vi "Test_C_RT_Path.vi"() -> ()   [LabVIEW 2021]
uses:
  CANsub_C.lvlib
  common/Typedefs/Bytes.ctl
  common/CANsub_Common.lvlib
  common/Typedefs/CAN_Frame.ctl
panel:
  out "ping length":i32
  out "encode mismatches":u32
  out "echo mismatches":u32
  out "error out":errorcluster
  out "peer close":bool
  out "decode errors":i32
  out "crc errors":u32
  out "frame mismatches":u32
  out "frames":i32
  # "Expected result when run"
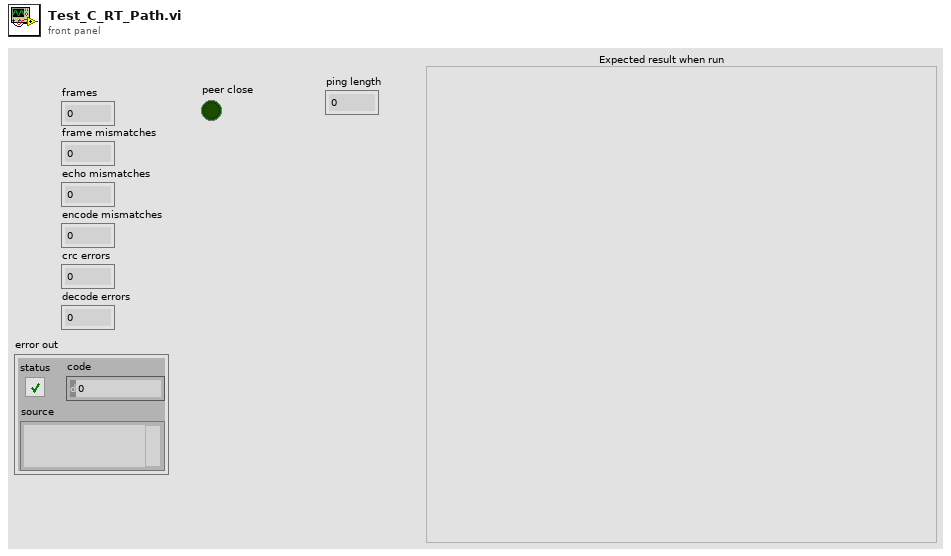
[diagram p1: front panel]
types:
  T1 = typedef "CANsub_Common.lvlib/CAN_Frame.ctl" = cluster{"t_dev":dbl, "id":u32, "ide":bool, "fdf":bool, "rtr":bool, "brs":bool, "esi":bool, "tx_ack":bool, "error":bool, "err type":u8, "dlc":u8, "data":T2}
  T2 = typedef "CANsub_Common.lvlib/Bytes.ctl" = u8[]
  T3 = typedef "CANsub_C.lvlib/C_RX_Buffers.ctl" = cluster{"t_dev":dbl[], "ws":u8[], "id":u32[], "flags":u16[], "hdlc":u8[], "dlc":u8[], "data len":u8[], "data":u8[], "ping":u8[]}
  T4 = typedef "CANsub_C.lvlib/C_Decode_Result.ctl" = cluster{"n frames":i32, "peer close":bool, "ping len":i32, "crc errors":u32, "decode errors":i32}
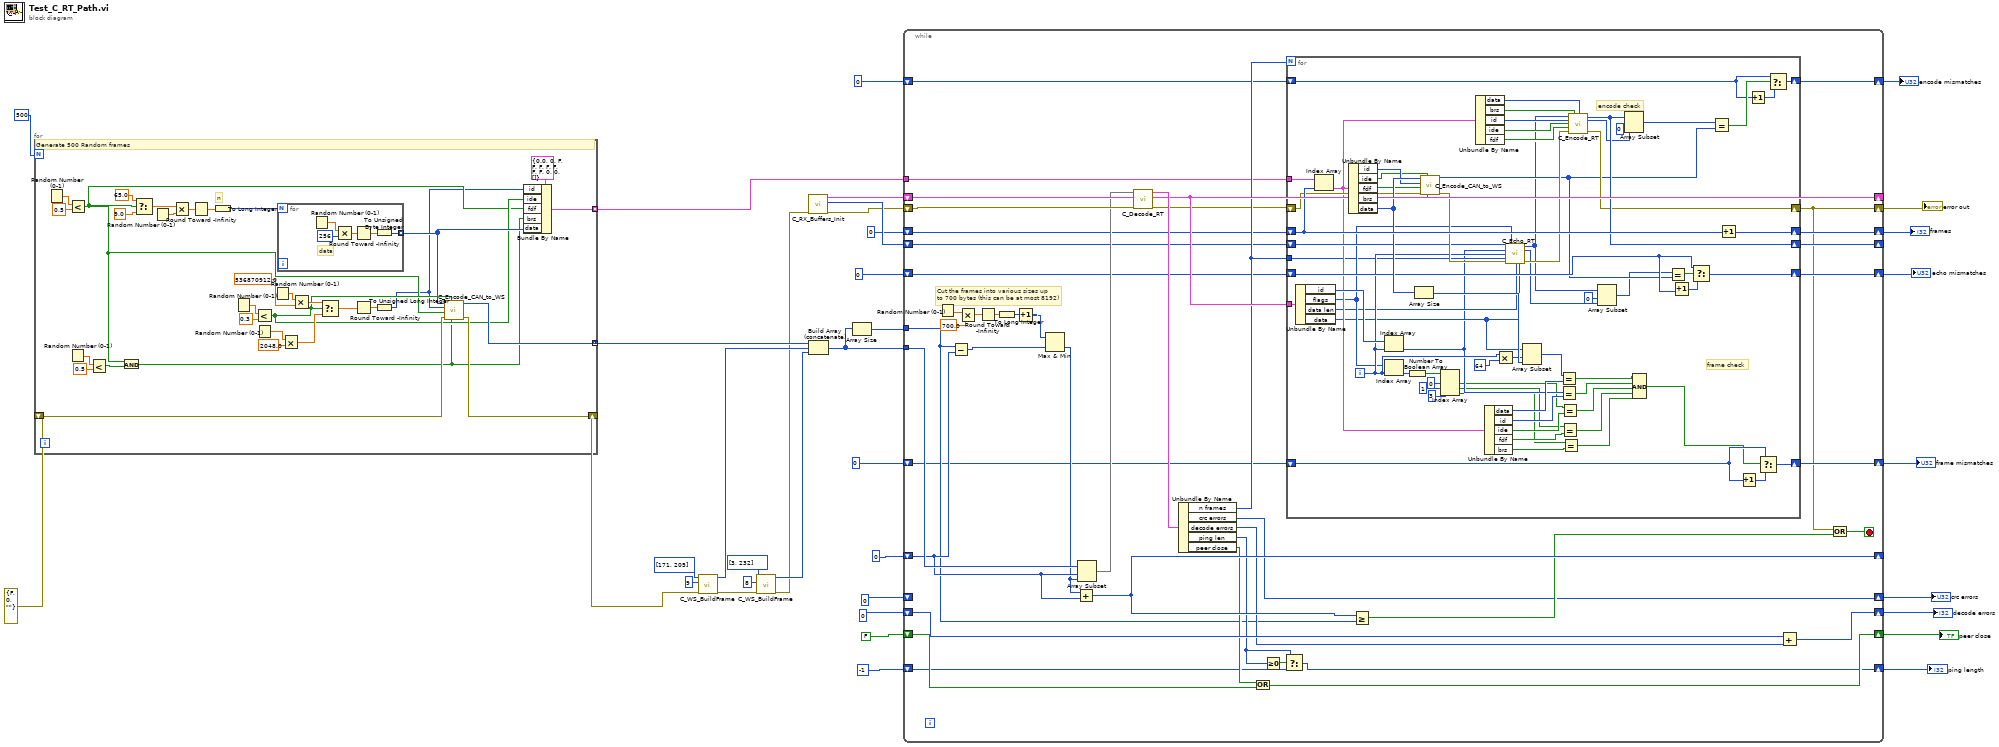
[diagram p0: block diagram]
diagram:
  n1 = for {
    N: 500 -> [_]
    shift-right: [w45] -> w14
    shift-left: errorcluster {"status"=FALSE, "code"=0, "source"=""} ("error constant") -> [w46]
    tunnel: [w47] -> w34 mode=concatenating
    tunnel: [w37] -> w2 mode=indexing
    # "n"
    # "Generate 500 Random frames"
    n2 = Random Number (0-1)() -> (number: 0 to 1=w68:dbl)
    n3 = Less?(x=w68, y=0.5) -> (x < y?=w40:bool)
    n4 = Random Number (0-1)() -> (number: 0 to 1=w65:dbl)
    n5 = Less?(x=w65, y=0.5) -> (x < y?=w64:bool)
    n6 = And(x=w40, y=w64) -> (x .and. y?=w39:bool)
    n7 = Select(t=65.0, s=w40, f=9.0) -> (s? t:f=w51:dbl)
    n8 = Random Number (0-1)() -> (number: 0 to 1=w50:dbl)
    n9 = Multiply(x=w51, y=w50) -> (x*y=w49:dbl)
    n10 = Round Toward -Infinity(1:w49) -> (0:w48:dbl)
    n11 = To Long Integer(number=w48) -> (32bit integer=w44:i32)
    n12 = Random Number (0-1)() -> (number: 0 to 1=w62:dbl)
    n13 = Less?(x=w62, y=0.3) -> (x < y?=w41:bool)
    n14 = Random Number (0-1)() -> (number: 0 to 1=w58:dbl)
    n15 = Random Number (0-1)() -> (number: 0 to 1=w61:dbl)
    n16 = for {
      N: w44 -> [_]
      tunnel: [w69] -> w42 mode=indexing
      # "data"
      n17 = Random Number (0-1)() -> (number: 0 to 1=w73:dbl)
      n18 = Multiply(x=w73, y=256) -> (x*y=w71:dbl)
      n19 = Round Toward -Infinity(1:w71) -> (0:w70:dbl)
      n20 = To Unsigned Byte Integer(number=w70) -> (unsigned 8bit integer=w69:u8)
    }
    n21 = Multiply(x=w58, y=2048.0) -> (x*y=w56:dbl)
    n22 = Multiply(x=w61, y=536870912.0) -> (x*y=w57:dbl)
    n23 = Select(t=w57, s=w41, f=w56) -> (s? t:f=w55:dbl)
    n24 = Round Toward -Infinity(1:w55) -> (0:w54:dbl)
    n25 = To Unsigned Long Integer(number=w54) -> (unsigned 32bit integer=w38:u32)
    n26 = call "C_Encode_CAN_to_WS.vi"("brs"=w39, "ide"=w41, "error in (no error)"=w46, "fdf"=w40, "id"=w38, "data"=w42) -> ("error out"=w45:errorcluster, "ws frame"=w47:u8[])  [unwired: 4 in]
    n27 = Bundle By Name(cluster=T1 {"t_dev"=0.0, "id"=0, "ide"=FALSE, "fdf"=FALSE, "rtr"=FALSE, "brs"=FALSE, "esi"=FALSE, "tx_ack"=FALSE, "error"=FALSE, "err type"=0, "dlc"=0, "data"=[]} ("CAN_Frame"), "id"=w38, "ide"=w41, "fdf"=w40, "brs"=w39, "data"=w42) -> (w37:T1)
  }
  n28 = call "C_WS_BuildFrame.vi"("error in (no error)"=w14, "opcode"=u8 9, "payload"=u8[] [171, 205]) -> ("error out"=w33:errorcluster, "frame"=w32:u8[])  [unwired: 7 in]
  n29 = call "C_WS_BuildFrame.vi"("error in (no error)"=w33, "opcode"=u8 8, "payload"=u8[] [3, 232]) -> ("error out"=w13:errorcluster, "frame"=w31:u8[])  [unwired: 7 in]
  n30 = call "C_RX_Buffers_Init.vi"("error in (no error)"=w13) -> ("error out"=w12:errorcluster, "tx"=w16:u8[], "buffers"=w17:T3)  [unwired: 7 in, 1 out]
  n31 = Build Array (concatenate)(w34, w32, w31) -> (w22:u8[])
  n32 = Array Size(array=w22) -> (size(s)=w1:i32)
  n33 = while {
    shift-right: [w107] -> _
    shift-left: 0 -> [w109]
    shift-right: [w101] -> w20
    shift-left: FALSE -> [w102]
    shift-right: [w91] -> w19
    shift-left: u32 0 -> [_]
    shift-right: [w103] -> w18
    shift-left: 0 -> [w104]
    shift-right: [w74] -> w21
    shift-left: w12 -> [w98]
    tunnel: w22 -> [w110]
    shift-right: [w89] -> _
    shift-left: w17 -> [w100]
    shift-right: [w78] -> _
    shift-left: w16 -> [w81]
    shift-right: [w80] -> w4
    shift-left: 0 -> [w86]
    shift-right: [w75] -> w11
    shift-left: u32 0 -> [w85]
    shift-right: [w76] -> w8
    shift-left: u32 0 -> [w84]
    shift-right: [w77] -> w10
    shift-left: u32 0 -> [w83]
    shift-right: [w92] -> w3
    shift-left: -1 -> [w95]
    tunnel: w2 -> [w79]
    tunnel: w1 -> [w88]
    stop <- w105 stop-if-true
    # "Cut the frames into various sizes up\nto 700 bytes (this can be at most 8192)"
    n34 = Random Number (0-1)() -> (number: 0 to 1=w117:dbl)
    n35 = Subtract(x=w88, y=w109) -> (x-y=w112:i32)
    n36 = Multiply(x=w117, y=700.0) -> (x*y=w115:dbl)
    n37 = Round Toward -Infinity(1:w115) -> (0:w114:dbl)
    n38 = To Long Integer(number=w114) -> (32bit integer=w113:i32)
    n39 = Increment(x=w113) -> (x+1=w111:i32)
    n40 = Max & Min(x=w111, y=w112) -> (min(x,y)=w108:i32)  [unwired: 1 out]
    n41 = Add(x=w108, y=w109) -> (x+y=w107:i32)
    n42 = Array Subset(array=w110, index=w109, length=w108) -> (w97:u8[])
    n43 = call "C_Decode_RT.vi"("error in (no error)"=w98, "buffers in"=w100, "bytes in"=w97) -> ("error out"=w82:errorcluster, "buffers out"=w89:T3, "result"=w99:T4)  [unwired: 6 in]
    n44 = Unbundle By Name(w99) -> ("n frames"=w87:i32, "crc errors"=w91:u32, "decode errors"=w90:i32, "ping len"=w93:i32, "peer close"=w96:bool)
    n45 = Or(x=w96, y=w102) -> (x .or. y?=w101:bool)
    n46 = Greater Or Equal To 0?(x=w93) -> (x >= 0?=w94:bool)
    n47 = Select(t=w93, s=w94, f=w95) -> (s? t:f=w92:i32)
    n48 = for {
      N: w87 -> [_]
      tunnel: w89 -> [w187]
      tunnel: w79 -> [w186]
      tunnel: w87 -> [w138]
      shift-right: [w185] -> w80
      shift-left: w86 -> [w184]
      shift-right: [w168] -> w74
      shift-left: w82 -> [w178]
      shift-right: [w169] -> w78
      shift-left: w81 -> [w160]
      shift-right: [w146] -> w75
      shift-left: w85 -> [w147]
      shift-right: [w151] -> w76
      shift-left: w84 -> [w150]
      shift-right: [w162] -> w77
      shift-left: w83 -> [w164]
      i -> [w144]
      # "encode check"
      # "frame check"
      n49 = Unbundle By Name(w187) -> ("id"=w176:u32[], "flags"=w141:u16[], "data len"=w140:u8[], "data"=w139:u8[])
      n50 = Index Array(array=w186, index=w184) -> (element=w143:T1)
      n51 = Unbundle By Name(w143) -> ("id"=w182:u32, "ide"=w181:bool, "fdf"=w180:bool, "brs"=w179:bool, "data"=w183:T2)
      n52 = Index Array(array=w176, index=w144) -> (element=w131:u32)
      n53 = Index Array(array=w141, index=w144) -> (element=w142:u16)
      n54 = Number To Boolean Array(number=w142) -> (Boolean array=w175:bool[])
      n55 = Array Size(array=w183) -> (size(s)=w177:i32)
      n56 = call "C_Encode_CAN_to_WS.vi"("brs"=w179, "ide"=w181, "error in (no error)"=w178, "fdf"=w180, "id"=w182, "data"=w183) -> ("error out"=w171:errorcluster, "ws frame"=w145:u8[])  [unwired: 4 in]
      n57 = Index Array(array=w175, index #1=0 ("index"), index #2=1 ("index"), index #3=3 ("index")) -> (element #1=w122:bool, element #2=w121:bool, element #3=w120:bool)
      n58 = Unbundle By Name(w143) -> ("data"=w159:T2, "brs"=w158:bool, "id"=w157:u32, "ide"=w156:bool, "fdf"=w155:bool)
      n59 = Unbundle By Name(w143) -> ("data"=w133:T2, "id"=w132:u32, "ide"=w130:bool, "fdf"=w129:bool, "brs"=w128:bool)
      n60 = Multiply(x=w144, y=64) -> (x*y=w153:i32)
      n61 = call "C_Echo_RT.vi"("tx in"=w160, "flags"=w141, "data len"=w140, "data"=w139, "new id"=w131, "index"=w144, "n frames"=w138, "error in (no error)"=w171) -> ("tx out"=w137:u8[], "length"=w136:i32, "error out"=w161:errorcluster)  [unwired: 5 in]
      n62 = Array Subset(array=w139, index=w153, length=w177) -> (w119:u8[])
      n63 = Equal?(x=w119, y=w133) -> (x = y?=w127:bool)
      n64 = Equal?(x=w131, y=w132) -> (x = y?=w126:bool)
      n65 = Equal?(x=w122, y=w130) -> (x = y?=w125:bool)
      n66 = Equal?(x=w121, y=w129) -> (x = y?=w124:bool)
      n67 = Equal?(x=w120, y=w128) -> (x = y?=w123:bool)
      n68 = call "C_Encode_RT.vi"("tx in"=w137, "brs"=w158, "data"=w159, "id"=w157, "ide"=w156, "fdf"=w155, "error in (no error)"=w161) -> ("tx out"=w169:u8[], "length"=w167:i32, "error out"=w168:errorcluster)  [unwired: 6 in]
      n69 = Array Subset(array=w137, index=0, length=w136) -> (w134:u8[])
      n70 = Array Subset(array=w169, index=0, length=w167) -> (w170:u8[])
      n71 = Compound Arithmetic op=AND(w127, w126, w125, w124, w123) -> (w118:bool)
      n72 = Equal?(x=w134, y=w145) -> (x = y?=w152:bool)
      n73 = Increment(x=w150) -> (x+1=w149:u32)
      n74 = Select(t=w150, s=w152, f=w149) -> (s? t:f=w151:u32)
      n75 = Equal?(x=w170, y=w145) -> (x = y?=w165:bool)
      n76 = Increment(x=w184) -> (x+1=w185:i32)
      n77 = Increment(x=w147) -> (x+1=w148:u32)
      n78 = Increment(x=w164) -> (x+1=w163:u32)
      n79 = Select(t=w147, s=w118, f=w148) -> (s? t:f=w146:u32)
      n80 = Select(t=w164, s=w165, f=w163) -> (s? t:f=w162:u32)
    }
    n81 = Greater Or Equal?(x=w107, y=w88) -> (x >= y?=w106:bool)
    n82 = Add(x=w104, y=w90) -> (x+y=w103:i32)
    n83 = Or(x=w74, y=w106) -> (x .or. y?=w105:bool)
  }
  "frames" <- w4
  "frame mismatches" <- w11
  "crc errors" <- w19
  "decode errors" <- w18
  "peer close" <- w20
  "error out" <- w21
  "echo mismatches" <- w8
  "encode mismatches" <- w10
  "ping length" <- w3
